vi "Tree to Variant.vi"(10 "Name":string="untitled", 11 "Variant Tree":variant) -> (3 "Variant":variant)   [LabVIEW 2013, in "OpenVariant.lvlib"]
uses:
  OpenVariant.lvlib
  TypeDescriptor/TypeDescriptor_GetName.vi
  TypeDescriptor/TypeDescriptor_GetType.vi
  Variant_EmptyCluster.vi
  TypeDescriptor/TypeDescriptor_GetPString.vi
  <vilib>/Utility/GetType.llb/Get Type Code from I16 Array And Pos.vi
  TypeDescriptor/TypeDescriptor_SetName.vi
  <vilib>/Utility/GetType.llb/TD_Create Cluster.vi
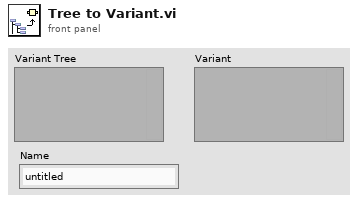
[diagram p1: front panel]
types:
  T1 = typedef "Type Enum.ctl" = enum8{"Void", "I8", "I16", "I32", "I64", "U8", "U16", "U32", "U64", "Single Float", "Double Float", "Extended Float", "Single Complex", "Double Complex", "Extended Complex", "Enum I8 NEVER", "Enum I16 NEVER", "Enum I32 NEVER", "Enum I64 NEVER", "Enum U8", "Enum U16", "Enum U32", "Enum U64", "Single Float With Unit", "Double Float With Unit", "Extended Float With Unit", "Single Complex With Unit", "Double Complex With Unit", "Extended Complex With Unit", "boolU16", "Boolean", "String", "Handle", "Path", "Picture", "C String", "Pascal String", "Tag", "SubString", "Array", "SubArray", "Cluster", "Numeric Cluster", "Variant", "LV Variant", "Measure Data (waveform)", "Refnum", "ExtData", "function", "Typedef", "Poly VI", "bad wire", "LabVIEW Class Instance"}
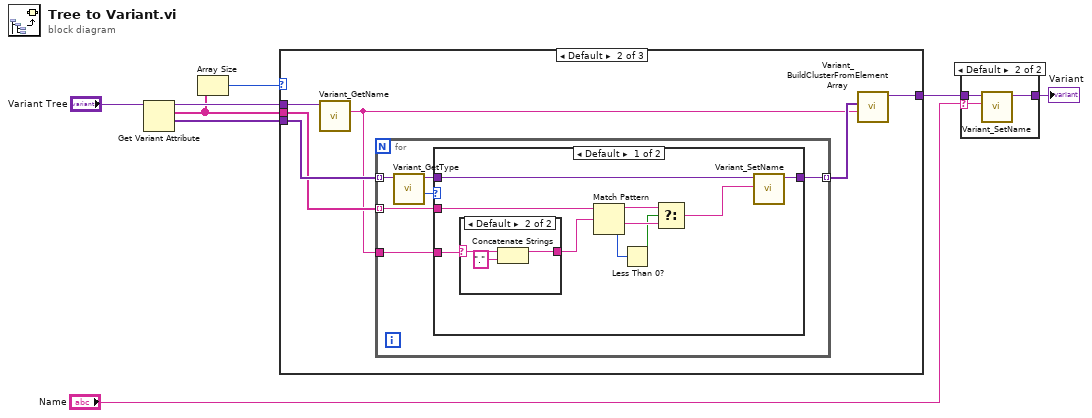
[diagram p0: block diagram]
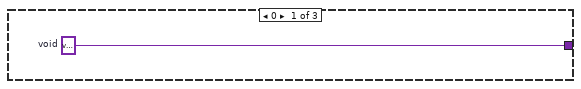
[diagram p3: hidden frame]
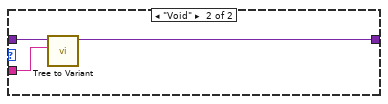
[diagram p5: hidden frame]
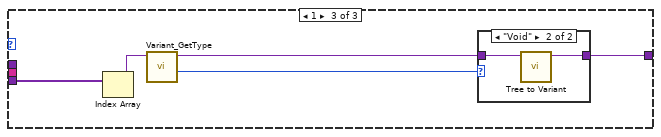
[diagram p6: hidden frame]
diagram:
  n1 = Get Variant Attribute(Variant="Variant Tree") -> (duplicate Variant=w8:variant, names=w5:string[], values=w4:variant[])  [unwired: 3 in, 1 out]
  n2 = Array Size(array=w5) -> (size(s)=w6:i32)
  n3 = case shown="Default" w6 {
    tunnel: w4 -> [_ w15 w43]
    tunnel: w5 -> [_ w11 _]
    tunnel: [w9 w12 w40] -> w2
    tunnel: w8 -> [_ w14 _]
    frame 0 {
      w9 = variant  # void
    }
    frame Default {
      n4 = call "Variant_GetName.vi"("Variant"=w14) -> ("Name"=w10:string)  [unwired: 8 in, 2 out]
      n5 = for {
        tunnel: w15 -> [w21] mode=indexing
        tunnel: [w18] -> w13 mode=indexing
        tunnel: w11 -> [w17] mode=indexing
        tunnel: w10 -> [w16]
        n6 = call "Variant_GetType.vi"("Variant"=w21) -> ("Type Enum"=w19:T1, "Variant dup"=w20:variant)  [unwired: 8 in, 1 out]
        n7 = case shown="Default" w19 {
          tunnel: w20 -> [w31 w38]
          tunnel: [w30 w37] -> w18
          tunnel: w17 -> [w28 w36]
          tunnel: w16 -> [w29 _]
          frame Default {
            n8 = case shown="Default" w29 {
              selector: w29 -> [w32 w35]
              tunnel: [w32 w33] -> w27
              frame "\u0000" {
              }
              frame Default {
                n9 = Concatenate Strings(w35, "." ("string")) -> (w33:string)
              }
            }
            n10 = Match Pattern(string=w28, regular expression=w27) -> (before substring=w26:string, after substring=w25:string, offset past match=w23:i32)  [unwired: 1 in, 1 out]
            n11 = Less Than 0?(x=w23) -> (x < 0?=w22:bool)
            n12 = Select(t=w26, s=w22, f=w25) -> (s? t:f=w24:string)
            n13 = call "Variant_SetName.vi"("Name"=w24, "Variant"=w31) -> ("Named Variant"=w30:variant)  [unwired: 9 in]
          }
          frame "Void" {
            n14 = call "Tree to Variant.vi"("Name"=w36, "Variant Tree"=w38) -> ("Variant"=w37:variant)  [unwired: 9 in]
          }
        }
      }
      n15 = call "Variant_BuildClusterFromElementArray.vi"("name"=w10, "Elements"=w13) -> ("Cluster"=w12:variant)  [unwired: 9 in]
    }
    frame 1 {
      n16 = Index Array(array=w43) -> (element=w39:variant)  [unwired: 1 in]
      n17 = call "Variant_GetType.vi"("Variant"=w39) -> ("Type Enum"=w41:T1, "Variant dup"=w42:variant)  [unwired: 8 in, 1 out]
      n18 = case shown="\"Void\"" w41 {
        tunnel: w42 -> [w44 w46]
        tunnel: [w44 w45] -> w40
        frame Default {
        }
        frame "Void" {
          n19 = call "Tree to Variant.vi"("Variant Tree"=w46) -> ("Variant"=w45:variant)  [unwired: 10 in]
        }
      }
    }
  }
  n20 = case shown="Default" "Name" {
    selector: "Name" -> [_ w48]
    tunnel: [w47 w50] -> w3
    tunnel: w2 -> [w47 w49]
    frame "" {
    }
    frame Default {
      n21 = call "Variant_SetName.vi"("Name"=w48, "Variant"=w49) -> ("Named Variant"=w50:variant)  [unwired: 9 in]
    }
  }
  "Variant" <- w3
